vi "Sous_VI_RT_trieur_balles.vi"(7 "Détection couleur IN":bool, 8 "error in (no error)":errorcluster, 9 "Nombre Balle IN":i32, 10 "Comteur IN":i32, 11 "Etat IN":T1) -> (0 "error out":errorcluster, 1 "Nombre Balle OUT":i32, 2 "Comteur OUT":i32, 3 "Etat OUT":T1, 4 "Indicateur de fin de process":bool, 5 "Détection couleur OUT":bool)   [LabVIEW 2018]
uses:
  enum_RT_trieur_Balles.ctl
panel:
  out "Couleur 4":bool
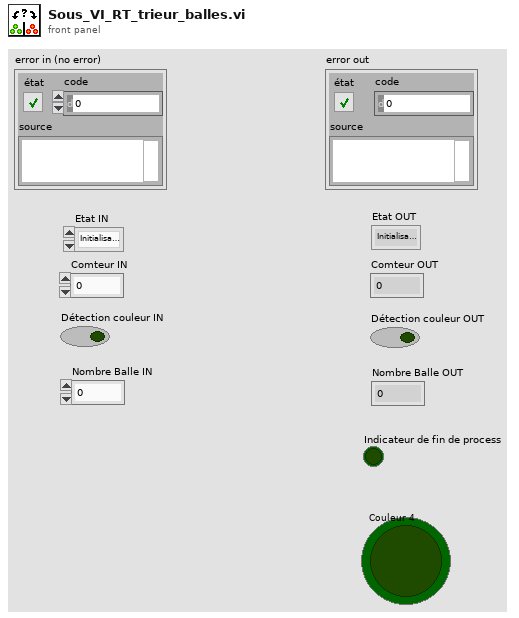
[diagram p1: front panel]
types:
  T1 = typedef "enum_RT_trieur_Balles.ctl" = enum16{"Initialisation", "Couleur", "Rotation1", "Rotation2", "Ouverture", "Fermeture"}
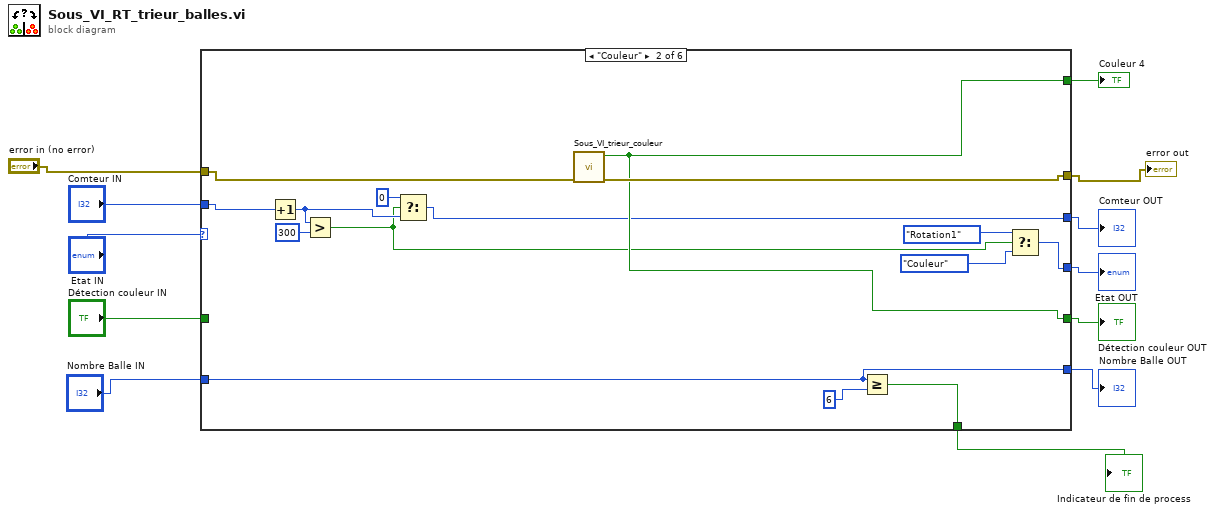
[diagram p0: block diagram]
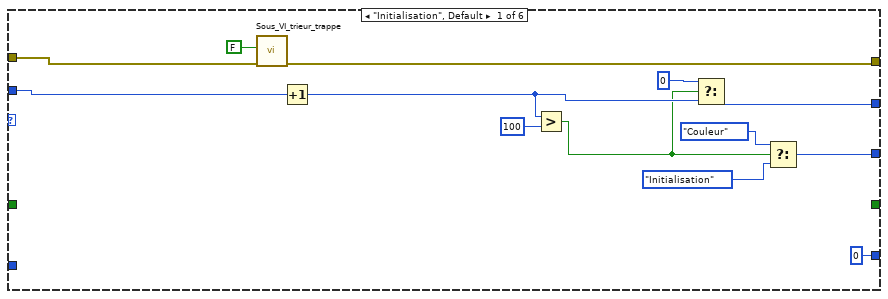
[diagram p2: hidden frame]
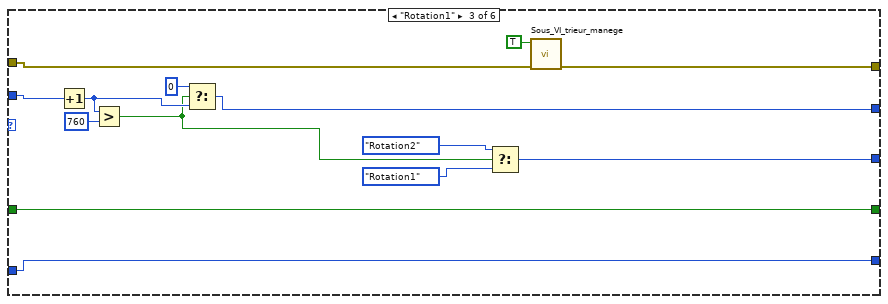
[diagram p3: hidden frame]
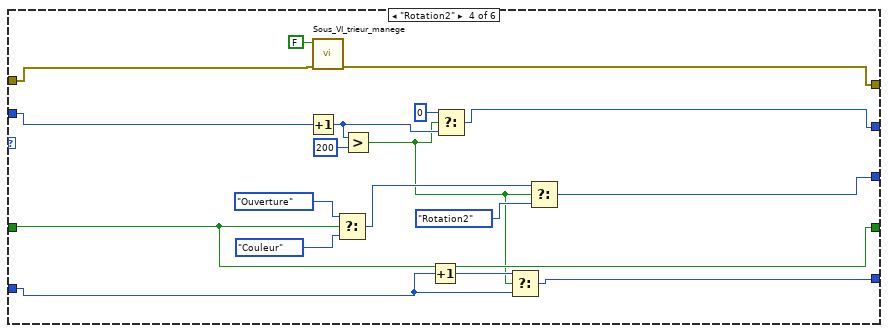
[diagram p4: hidden frame]
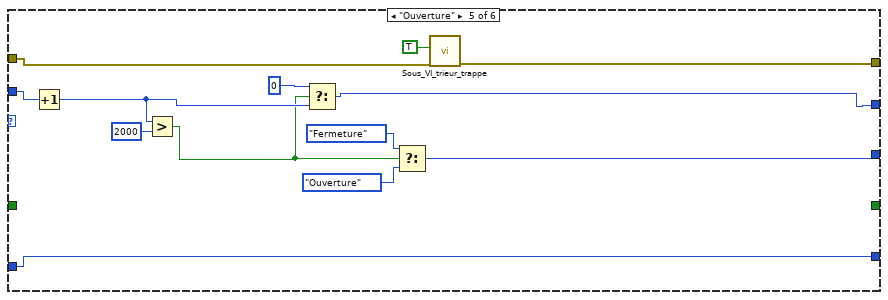
[diagram p5: hidden frame]
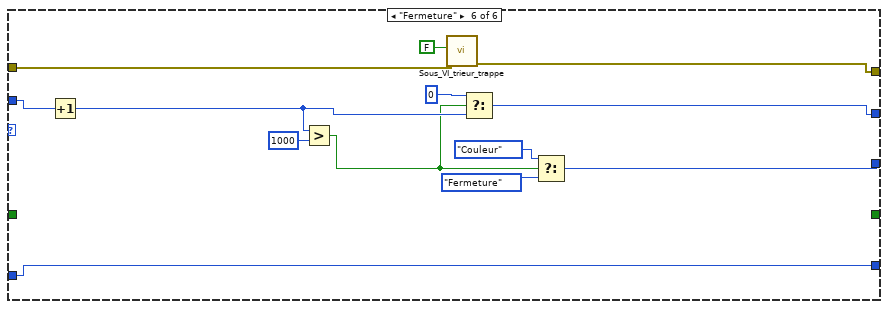
[diagram p6: hidden frame]
diagram:
  n1 = case shown="\"Couleur\"" "Etat IN" {
    tunnel: [w20 w40 w46 w63 w76 w89] -> w4
    tunnel: [w19 w27 w45 w64 w77 w90] -> w9
    tunnel: [w18 w34 w47 w65 w78 w91] -> w6
    tunnel: [_ w38 w48 w66 _ _] -> w7
    tunnel: "error in (no error)" -> [w17 w39 w50 w68 w80 w93]
    tunnel: "Comteur IN" -> [w16 w28 w49 w67 w79 w92]
    tunnel: "Détection couleur IN" -> [_ _ w48 w66 _ _]
    tunnel: [_ w38 _ _ _ _] -> w8
    tunnel: "Nombre Balle IN" -> [_ w35 w41 w57 w73 w86]
    tunnel: [_ w36 _ _ _ _] -> w2
    tunnel: [0 ("Nombre Balle IN") w35 w41 w58 w73 w86] -> w1
    frame "Initialisation", Default {
      n2 = call "Sous_VI_trieur_trappe.vi"("error in (no error)"=w17, "Ouvrir"=FALSE) -> ("error out"=w20:errorcluster)  [unwired: 9 in]
      n3 = Increment(x=w16) -> (x+1=w23:i32)
      n4 = Greater?(x=w23, y=100) -> (0:w22:bool)
      n5 = Select(t=0 ("cas vrai"), s=w22, f=w23) -> (s? t:f=w19:i32)
      n6 = Select(t=enum_RT_trieur_Balles."Couleur", s=w22, f=enum_RT_trieur_Balles."Initialisation") -> (s? t:f=w18:T1)
    }
    frame "Couleur" {
      n7 = Increment(x=w28) -> (x+1=w30:i32)
      n8 = Greater?(x=w30, y=300) -> (0:w26:bool)
      n9 = Select(t=0 ("cas vrai"), s=w26, f=w30) -> (s? t:f=w27:i32)
      n10 = call "Sous_VI_trieur_couleur.vi"("error in (no error)"=w39) -> ("error out"=w40:errorcluster, "Couleur"=w38:bool)  [unwired: 7 in]
      n11 = Greater Or Equal?(x=w35, y=6) -> (x >= y?=w36:bool)
      n12 = Select(t=enum_RT_trieur_Balles."Rotation1", s=w26, f=enum_RT_trieur_Balles."Couleur") -> (s? t:f=w34:T1)
    }
    frame "Rotation1" {
      n13 = Increment(x=w49) -> (x+1=w53:i32)
      n14 = Greater?(x=w53, y=760) -> (0:w51:bool)
      n15 = Select(t=0 ("cas vrai"), s=w51, f=w53) -> (s? t:f=w45:i32)
      n16 = Select(t=enum_RT_trieur_Balles."Rotation2", s=w51, f=enum_RT_trieur_Balles."Rotation1") -> (s? t:f=w47:T1)
      n17 = call "Sous_VI_trieur_manege.vi"("error in (no error)"=w50, "ON/OFF"=TRUE) -> ("error out"=w46:errorcluster)  [unwired: 9 in]
    }
    frame "Rotation2" {
      n18 = Increment(x=w67) -> (x+1=w71:i32)
      n19 = call "Sous_VI_trieur_manege.vi"("error in (no error)"=w68, "ON/OFF"=FALSE) -> ("error out"=w63:errorcluster)  [unwired: 9 in]
      n20 = Select(t=enum_RT_trieur_Balles."Ouverture", s=w66, f=enum_RT_trieur_Balles."Couleur") -> (s? t:f=w69:T1)
      n21 = Greater?(x=w71, y=200) -> (0:w55:bool)
      n22 = Increment(x=w57) -> (x+1=w56:i32)
      n23 = Select(t=0 ("cas vrai"), s=w55, f=w71) -> (s? t:f=w64:i32)
      n24 = Select(t=w56, s=w55, f=w57) -> (s? t:f=w58:i32)
      n25 = Select(t=w69, s=w55, f=enum_RT_trieur_Balles."Rotation2") -> (s? t:f=w65:T1)
    }
    frame "Ouverture" {
      n26 = Increment(x=w79) -> (x+1=w83:i32)
      n27 = Greater?(x=w83, y=2000) -> (0:w82:bool)
      n28 = Select(t=0 ("cas vrai"), s=w82, f=w83) -> (s? t:f=w77:i32)
      n29 = Select(t=enum_RT_trieur_Balles."Fermeture", s=w82, f=enum_RT_trieur_Balles."Ouverture") -> (s? t:f=w78:T1)
      n30 = call "Sous_VI_trieur_trappe.vi"("error in (no error)"=w80, "Ouvrir"=TRUE) -> ("error out"=w76:errorcluster)  [unwired: 9 in]
    }
    frame "Fermeture" {
      n31 = Increment(x=w92) -> (x+1=w96:i32)
      n32 = Greater?(x=w96, y=1000) -> (0:w95:bool)
      n33 = call "Sous_VI_trieur_trappe.vi"("error in (no error)"=w93, "Ouvrir"=FALSE) -> ("error out"=w89:errorcluster)  [unwired: 9 in]
      n34 = Select(t=0 ("cas vrai"), s=w95, f=w96) -> (s? t:f=w90:i32)
      n35 = Select(t=enum_RT_trieur_Balles."Couleur", s=w95, f=enum_RT_trieur_Balles."Fermeture") -> (s? t:f=w91:T1)
    }
  }
  "Comteur OUT" <- w9
  "Couleur 4" <- w8
  "Détection couleur OUT" <- w7
  "Etat OUT" <- w6
  "error out" <- w4
  "Nombre Balle OUT" <- w1
  "Indicateur de fin de process" <- w2
